vi "Kinect - Weak detect (SubVI).vi"(7 "error in":errorcluster, 10 "Array of Joint Positions In":dbl[][](array[numeric])) -> (0 "error out":errorcluster, 2 "Weak detect":bool, 3 "Array of Joint Positions Out":dbl[][](array[numeric]))   [LabVIEW 2014]
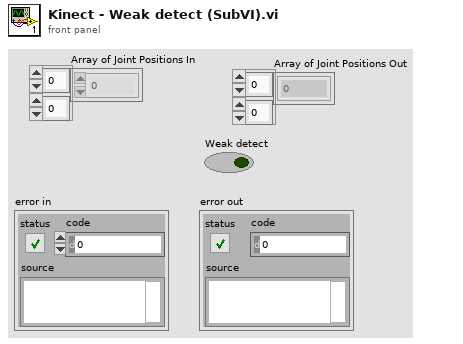
[diagram p1: front panel]
types:
  T1 = enum16{"hip centre", "spine", "shoulder centre", "head", "shoulder left", "elbow left", "wrist left", "hand left", "shoulder right", "elbow right", "wrist right", "hand right", "hip left", "knee left", "ankle left", "foot left", "hip right", "knee right", "ankle right", "foot right"}
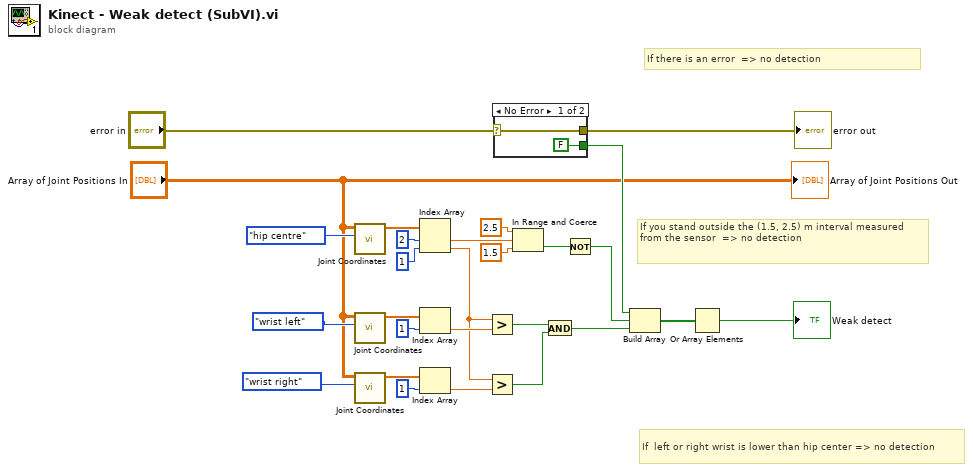
[diagram p0: block diagram]
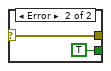
[diagram p2: hidden frame]
diagram:
  # "If there is an error  => no detection"
  # "If you stand outside the (1.5, 2.5) m interval measured from the sensor  => no detection"
  # "If  left or right wrist is lower than hip center => no detection"
  n1 = call <vilib>:"Joint Coordinates.vi"("Joint 1"=T1."hip centre", "Array of Joint Positions"="Array of Joint Positions In") -> ("Joint Coordinates"=w24:dbl[])  [unwired: 8 in, 1 out]
  n2 = call <vilib>:"Joint Coordinates.vi"("Joint 1"=T1."wrist left", "Array of Joint Positions"="Array of Joint Positions In") -> ("Joint Coordinates"=w18:dbl[])  [unwired: 8 in, 1 out]
  n3 = call <vilib>:"Joint Coordinates.vi"("Joint 1"=T1."wrist right", "Array of Joint Positions"="Array of Joint Positions In") -> ("Joint Coordinates"=w13:dbl[])  [unwired: 8 in, 1 out]
  n4 = Index Array(array=w24, index #1=2 ("index"), index #2=1 ("index")) -> (element #1=w2:dbl, element #2=w11:dbl)
  n5 = Index Array(array=w18, index=1) -> (element=w17:dbl)
  n6 = Index Array(array=w13, index=1) -> (element=w12:dbl)
  n7 = Greater?(x=w11, y=w17) -> (0:w10:bool)
  n8 = Greater?(x=w11, y=w12) -> (0:w9:bool)
  n9 = case shown="No Error" "error in" {
    selector: "error in" -> [w29 w30]
    tunnel: [FALSE TRUE] -> w16
    tunnel: [w29 w30] -> w27
    frame No Error {
    }
    frame Error {
    }
  }
  "error out" <- w27
  n10 = In Range and Coerce(upper limit=2.5 ("lower limit"), x=w2, lower limit=1.5 ("upper limit")) -> (In Range?=w22:bool)  [unwired: 1 out]
  n11 = And(x=w10, y=w9) -> (x .and. y?=w8:bool)
  n12 = Not(x=w22) -> (.not. x?=w5:bool)
  n13 = Build Array(w16, w5, w8) -> (w7:bool[])
  n14 = Or Array Elements(Boolean array=w7) -> (logical OR=→"Weak detect":bool)
  "Array of Joint Positions Out" <- "Array of Joint Positions In"
